vi "Not A Host Key Database.vi"(1 "host key database":T1) -> (0 "Not a Host Key Database?":bool)   [LabVIEW 2017, in "libssh2.lvlib"]
doc: "Returns TRUE if <B>host key database</B> is not a host key database. Otherwise, FALSE."
uses:
  libssh2.lvlib
  Host Key Database Refnum.ctl
  Host Key Database Refnum Data.ctl
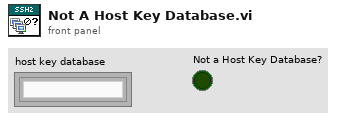
[diagram p1: front panel]
types:
  T1 = typedef "libssh2.lvlib/Host Key Database Refnum.ctl" = refnum<k1>
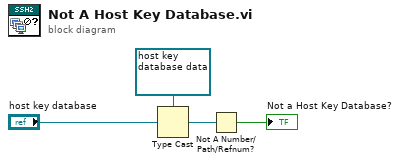
[diagram p0: block diagram]
diagram:
  n1 = Type Cast(type=refnum<data-value> refnum ("data value reference"), x="host key database") -> (*(type *) &x=w2:refnum<data-value>)
  n2 = Not A Number/Path/Refnum?(number/path/refnum=w2) -> (NaN/Path/Refnum?=→"Not a Host Key Database?":bool)
